vi "RemoteVI Check JSON String.vi"() -> (4 "labels":string[](array[string]), 6 "expected":string[](array[string]), 8 "actual":string[](array[string]), 10 "failures":i32)   [LabVIEW 2020]
doc: "Test support, generated by tests/caraya/build.py from tests/vectors/text.json (jsonStrings) - do not edit. Calls RemoteVI JSON String.vi once per vector: text is the vector's UTF-16 code units, json is compared as the string literal it is. Outputs, one element per vector: labels (the vector's name), expected (rendered from the vector), actual (the VI's result rendered the same way), and failures, the number of vectors whose expected and actual differ."
uses:
  source/RemoteVI.lvlib
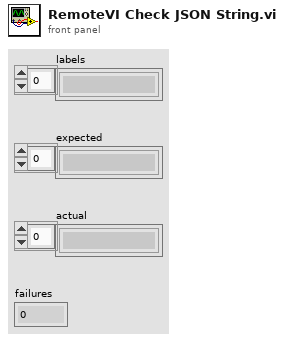
[diagram p1: front panel]
types:
  T1 = cluster{"name":string, "text":u16[], "expect":string}[]
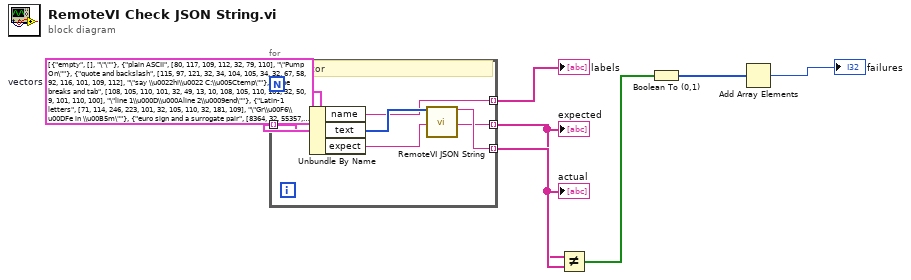
[diagram p0: block diagram]
diagram:
  w1 = T1 [{"name"="empty", "text"=[], "expect"="\"\""}, {"name"="plain ASCII", "text"=[80, 117, 109, 112, 32, 79, 110], "expect"="\"Pump On\""}, {"name"="quote and backslash", "text"=[115, 97, 121, 32, 34, 104, 105, 34, 32, 67, 58, 92, 116, 101, 109, 112], "expect"="\"say \\u0022hi\\u0022 C:\\u005Ctemp\""}, {"name"="line breaks and tab", "text"=[108, 105, 110, 101, 32, 49, 13, 10, 108, 105, 110, 101, 32, 50, 9, 101, 110, 100], "expect"="\"line 1\\u000D\\u000Aline 2\\u0009end\""}, {"name"="Latin-1 letters", "text"=[71, 114, 246, 223, 101, 32, 105, 110, 32, 181, 109], "expect"="\"Gr\\u00F6\\u00DFe in \\u00B5m\""}, {"name"="euro sign and a surrogate pair", "text"=[8364, 32, 55357, 56832], "expect"="\"\\u20AC \\uD83D\\uDE00\""}, {"name"="DEL and tilde", "text"=[126, 127], "expect"="\"~\\u007F\""}]  # vectors
  n1 = for {
    tunnel: w1 -> [w8] mode=indexing
    tunnel: [w9] -> w2 mode=indexing
    tunnel: [w11] -> w3 mode=indexing
    tunnel: [w12] -> w4 mode=indexing
    # "One vector"
    n2 = Unbundle By Name(w8) -> ("name"=w9:string, "text"=w10:u16[], "expect"=w11:string)
    n3 = call "RemoteVI JSON String.vi"("text"=w10) -> ("json"=w12:string)  [unwired: 14 in]
  }
  "labels" <- w2
  "expected" <- w3
  "actual" <- w4
  n4 = Not Equal?(x=w3, y=w4) -> (x != y?=w5:bool[])
  n5 = Boolean To (0,1)(Boolean=w5) -> (0, 1=w6:i16[])
  n6 = Add Array Elements(numeric array=w6) -> (sum=→"failures":i16)
